vi "RemoteVI Find Popups.vi"(0 "panel hWnd":u64, 11 "error in":errorcluster) -> (4 "popups":T1(array[cluster]), 15 "error out":errorcluster)   [LabVIEW 2020, in "RemoteVI.lvlib"]
doc: "Lists the visible popup windows of the panel's process (LabVIEW's own, or another LabVIEW's for a window target) - ring and enum menus (class LVMenuWnd), and other captionless WS_POPUP windows such as shortcut menus and combo box drop-downs - which FP.Get Image does not include. It walks the top-level windows in Z order with FindWindowExW(0, previous, NULL, NULL) from the top down to the panel's owner (user32 GetWindow.vi GW_OWNER - LabVIEW's hidden frame window LVFrame, which owns the panels and the popups; an owned window is always above its owner and a topmost popup above every non-topmost window, so no popup lies below it) or to the end when the panel has no owner - the whole walk took 61 ms with 860 top-level windows on the desktop, the walk down to LVFrame a few ms (measured), keeps those whose process is LabVIEW's (GetWindowThreadProcessId = GetCurrentProcessId) and that are not panel hWnd, and asks RemoteVI Window Popup Info.vi about each. Win32 calls only, no VI Server, so it runs while an open menu holds LabVIEW's UI thread in its modal loop. Meant to run on every server loop iteration."
uses:
  RemoteVI.lvlib
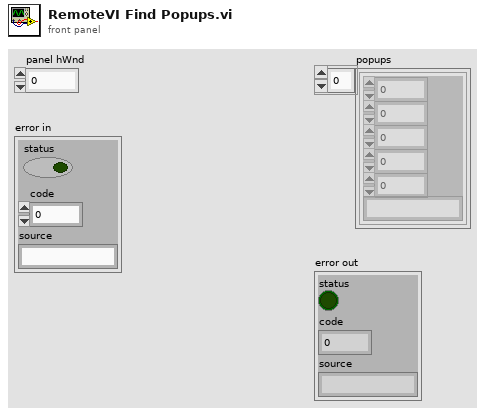
[diagram p1: front panel]
types:
  T1 = cluster{"hwnd":u64, "x":i32, "y":i32, "w":i32, "h":i32, "class":string}[]
  T2 = cluster{"hwnd":u64, "x":i32, "y":i32, "w":i32, "h":i32, "class":string}
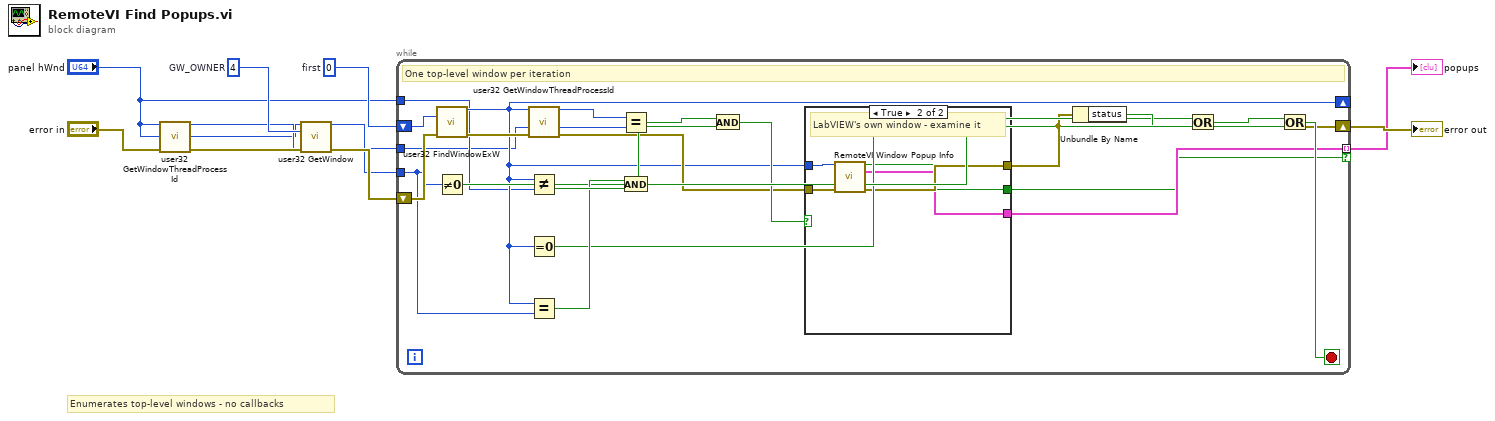
[diagram p0: block diagram]
diagram:
  w8 = u32 4  # GW_OWNER
  w7 = u64 0  # first
  # "Enumerates top-level windows - no callbacks"
  n1 = call "user32 GetWindowThreadProcessId.vi"("hWnd"="panel hWnd", "error in"="error in") -> ("process ID"=w5:u32, "error out"=w6:errorcluster)  [unwired: 11 in, 1 out]
  n2 = call "user32 GetWindow.vi"("hWnd"="panel hWnd", "uCmd"=w8, "error in"=w6) -> ("window"=w9:u64, "error out"=w10:errorcluster)  [unwired: 11 in]
  n3 = while {
    tunnel: "panel hWnd" -> [w12]
    shift-right: [w15] -> _
    shift-left: w7 -> [w14]
    tunnel: w5 -> [w11]
    tunnel: w9 -> [w13]
    shift-right: [w17] -> w4
    shift-left: w10 -> [w16]
    tunnel: [w25] -> w3 mode=indexing if=w24
    stop <- w32 stop-if-true
    # "One top-level window per iteration"
    n4 = call "user32 FindWindowExW.vi"("hWndChildAfter"=w14, "error in"=w16) -> ("hWnd"=w15:u64, "error out"=w18:errorcluster)  [unwired: 12 in]
    n5 = Not Equal To 0?(x=w13) -> (x != 0?=w29:bool)
    n6 = call "user32 GetWindowThreadProcessId.vi"("hWnd"=w15, "error in"=w18) -> ("process ID"=w19:u32, "error out"=w20:errorcluster)  [unwired: 11 in, 1 out]
    n7 = Not Equal?(x=w15, y=w12) -> (x != y?=w22:bool)
    n8 = Equal To 0?(x=w15) -> (x = 0?=w26:bool)
    n9 = Equal?(x=w15, y=w13) -> (x = y?=w28:bool)
    n10 = Equal?(x=w19, y=w11) -> (x = y?=w21:bool)
    n11 = And(x=w28, y=w29) -> (x .and. y?=w30:bool)
    n12 = And(x=w21, y=w22) -> (x .and. y?=w23:bool)
    n13 = case shown="True" w23 {
      tunnel: w15 -> [_ w34]
      tunnel: w20 -> [w33 w35]
      tunnel: [w33 w38] -> w17
      tunnel: [_ w36] -> w24
      tunnel: [_ w37] -> w25
      frame False {
        # "Another process or the panel"
      }
      frame True {
        # "LabVIEW's own window - examine it"
        n14 = call "RemoteVI Window Popup Info.vi"("hWnd"=w34, "error in"=w35) -> ("popup?"=w36:bool, "window"=w37:T2, "error out"=w38:errorcluster)  [unwired: 11 in]
      }
    }
    n15 = Unbundle By Name(w17) -> ("status"=w27:bool)
    n16 = Or(x=w26, y=w27) -> (x .or. y?=w31:bool)
    n17 = Or(x=w31, y=w30) -> (x .or. y?=w32:bool)
  }
  "popups" <- w3
  "error out" <- w4
